vi "SQL_Search_Drivername.vi"(6 "Client Name (MSOLEDBSQL)":string="MSOLEDBSQL", 8 "error in (no error)":errorcluster caption="Fehler (Eingang, kein Fehler)") -> (0 "error out":errorcluster caption="Fehler (Ausgang)", 1 "Driver":string[](array[string]) caption="Alle ODBC Driver", 2 "found?":bool, 3 "Client Name":string)   [LabVIEW 2024, in "DB-Tool.lvlib"]
doc: "Es wird in der Windows-Registry nach dem angegebenen SQL-OLEDB-Provider gesucht.\nStandardmäßig wird nach \"<b>MSOLEDBSQL</b>\" gesucht, um einen installierten Microsoft SQL Server OLE DB Treiber zu finden.\n\n<b>Wichtig:</b>\nDer <b>SQL Server Native Client (SQLNCLI)</b> gilt als veraltet und sollte für neue Projekte nicht mehr verwendet werden.\nMicrosoft empfiehlt für Neuentwicklungen den aktuellen <b>Microsoft OLE DB Driver for SQL Server (MSOLEDBSQL)</b>.\n\n\nDer aktuelle Treiber kann hier heruntergeladen werden:\nhttps://learn.microsoft.com/en-us/sql/connect/oledb/download-oledb-driver-for-sql-server?view=sql-server-ver17\nMicrosoft OLE DB Driver for SQL Server herunterladen\n\nDas VI durchsucht die Registry nach verfügbaren SQL-OLEDB-Treibern und liefert den gefundenen Providernamen zurück.\nDadurch kann die Anwendung verschiedene installierte Treiberversionen automatisch erkennen, Beispielsweise: \n MSOLEDBSQL\n MSOLEDBSQL18\n MSOLEDBSQL19\n\nWird kein passender Treiber gefunden, wird der Ausgang <b>found?</b> auf FALSE gesetzt.\n\nEingänge:\n- Client Name: Name des gesuchten SQL/OLEDB-Clients (Standard wird nach MSOLEDBSQL gesucht).\n- error in: Hat keinen Einfluss über die Funktion.\n\nAusgänge:\n- Driver: Gefundener Treibername.\n- found?: TRUE, wenn ein passender Treiber gefunden wurde."
uses:
  <vilib>/registry/registry.llb/Registry RtKey.ctl
  <vilib>/registry/registry.llb/Registry SAM.ctl
  <vilib>/regexp/Match Regular Expression.xnode
  DB-Tool.lvlib
panel:
  # "Alt, sollte nicht mehr verwendet werden\nSQL Server Native Client\n\nNeu MSOLEDBSQL \n(sucht nach dem Treiber z.b. MSOLEDBSQL19.1)"
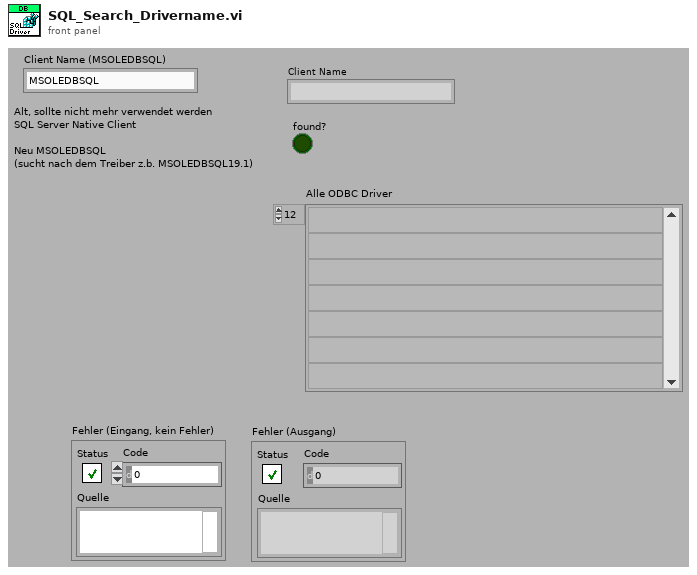
[diagram p1: front panel]
types:
  T1 = typedef "Registry SAM.ctl" = enum32{"KEY_QUERY_VALUE", "KEY_SET_VALUE", "KEY_CREATE_SUB_KEY", "KEY_ENUMERATE_SUB_KEYS", "KEY_NOTIFY", "KEY_CREATE_LINK", "KEY_READ", "KEY_WRITE", "KEY_ALL_ACCESS", "KEY_READ | KEY_WRITE"}
  T2 = typedef "Registry RtKey.ctl" = enum32{"HKEY_CLASSES_ROOT", "HKEY_CURRENT_USER", "HKEY_LOCAL_MACHINE", "HKEY_USERS", "HKEY_PERFORMANCE_DATA", "HKEY_CURRENT_CONFIG", "HKEY_DYN_DATA"}
  T3 = typedef "Registry refnum.ctl" = refnum<k1>
  T4 = cluster{"numSubKeys":i32, "maxSubKeyLen":i32, "maxSubKeyClassLen":i32}
  T5 = cluster{"numValues":i32, "maxValueNameLen":i32, "maxValueDataLen":i32}
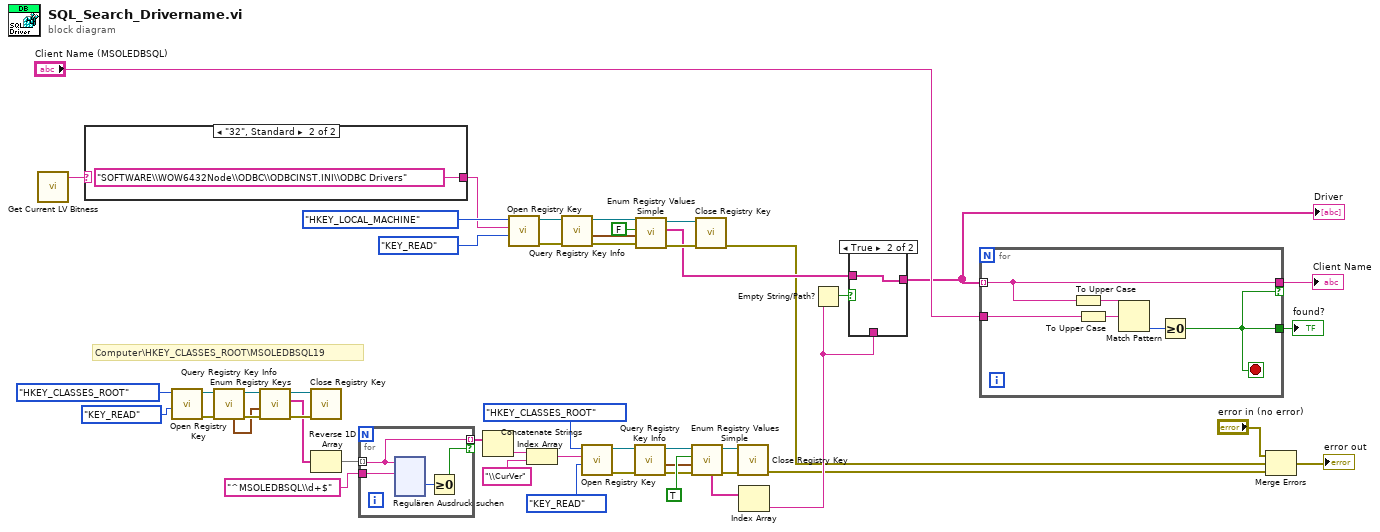
[diagram p0: block diagram]
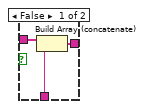
[diagram p2: hidden frame]
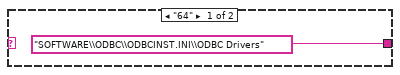
[diagram p3: hidden frame]
diagram:
  # "Computer\\HKEY_CLASSES_ROOT\\MSOLEDBSQL19"
  n1 = call <vilib>:"Get Current LV Bitness.vi"() -> ("bitness"=w45:string)  [unwired: 11 in]
  n2 = case shown="\"32\", Standard" w45 {
    tunnel: ["SOFTWARE\\ODBC\\ODBCINST.INI\\ODBC Drivers" ("subkey") "SOFTWARE\\WOW6432Node\\ODBC\\ODBCINST.INI\\ODBC Drivers" ("subkey")] -> w31
    frame "64" {
    }
    frame "32", Default {
    }
  }
  n3 = call <vilib>:"Open Registry Key.vi"("security access mask (KEY_READ | KEY_WRITE)"=Registry_SAM."KEY_READ", "root key (HKEY_LOCAL_MACHINE)"=Registry_RtKey."HKEY_CLASSES_ROOT") -> ("error out"=w33:errorcluster, "refnum out"=w35:T3)  [unwired: 8 in]
  n4 = call <vilib>:"Query Registry Key Info.vi"("error in (no error)"=w33, "refnum"=w35) -> ("error out"=w28:errorcluster, "refnum out"=w21:T3, "subkey info"=w22:T4)  [unwired: 5 in, 2 out]
  n5 = call <vilib>:"Enum Registry Keys.vi"("error in (no error)"=w28, "subkey info"=w22, "refnum"=w21) -> ("error out"=w30:errorcluster, "subkeys"=w27:string[], "refnum out"=w20:T3)  [unwired: 6 in]
  n6 = call <vilib>:"Close Registry Key.vi"("error in (no error)"=w30, "refnum"=w20) -> ()  [unwired: 5 in, 1 out]
  n7 = Reverse 1D Array(array=w27) -> (reversed array=w26:string[])
  n8 = for {
    tunnel: w26 -> [w55] mode=indexing
    tunnel: [w55] -> w25 mode=indexing if=w54
    tunnel: "^MSOLEDBSQL\\d+$" ("Regulärer Ausdruck") -> [w53]
    n9 = xnode "Regulären Ausdruck suchen"("Eingangs-String"=w55, "Regulärer Ausdruck"=w53) -> ("Offset nach Übereinstimmung"=w56:i32)  [unwired: 4 in, 4 out]
    n10 = Greater Or Equal To 0?(x=w56) -> (x >= 0?=w54:bool)
  }
  n11 = Index Array(array=w25) -> (element=w8:string)  [unwired: 1 in]
  n12 = call <vilib>:"Open Registry Key.vi"("security access mask (KEY_READ | KEY_WRITE)"=Registry_SAM."KEY_READ", "subkey"=w31, "root key (HKEY_LOCAL_MACHINE)"=Registry_RtKey."HKEY_LOCAL_MACHINE") -> ("error out"=w41:errorcluster, "refnum out"=w37:T3)  [unwired: 7 in]
  n13 = Concatenate Strings(w8, "\\CurVer" ("String")) -> (w7:string)
  n14 = call <vilib>:"Query Registry Key Info.vi"("error in (no error)"=w41, "refnum"=w37) -> ("error out"=w42:errorcluster, "value info"=w36:T5, "refnum out"=w29:T3)  [unwired: 5 in, 2 out]
  n15 = call <vilib>:"Open Registry Key.vi"("security access mask (KEY_READ | KEY_WRITE)"=Registry_SAM."KEY_READ", "subkey"=w7, "root key (HKEY_LOCAL_MACHINE)"=Registry_RtKey."HKEY_CLASSES_ROOT") -> ("error out"=w18:errorcluster, "refnum out"=w16:T3)  [unwired: 7 in]
  n16 = call <vilib>:"Query Registry Key Info.vi"("error in (no error)"=w18, "refnum"=w16) -> ("error out"=w9:errorcluster, "value info"=w13:T5, "refnum out"=w15:T3)  [unwired: 5 in, 2 out]
  n17 = call <vilib>:"Enum Registry Values Simple.vi"("error in (no error)"=w42, "value info"=w36, "retrieve data? (F)"=FALSE, "refnum"=w29) -> ("error out"=w40:errorcluster, "values"=w24:string[], "refnum out"=w39:T3)  [unwired: 2 in, 3 out]
  n18 = call <vilib>:"Enum Registry Values Simple.vi"("error in (no error)"=w9, "value info"=w13, "retrieve data? (F)"=TRUE, "refnum"=w15) -> ("error out"=w10:errorcluster, "refnum out"=w11:T3, "String/Binary data"=w12:string[])  [unwired: 2 in, 3 out]
  n19 = call <vilib>:"Close Registry Key.vi"("error in (no error)"=w40, "refnum"=w39) -> ("error out"=w2:errorcluster)  [unwired: 5 in]
  n20 = call <vilib>:"Close Registry Key.vi"("error in (no error)"=w10, "refnum"=w11) -> ("error out"=w1:errorcluster)  [unwired: 5 in]
  n21 = Index Array(array=w12) -> (element=w4:string)  [unwired: 1 in]
  n22 = Empty String/Path?(string/path=w4) -> (empty?=w3:bool)
  n23 = case shown="True" w3 {
    tunnel: w24 -> [w176 w177]
    tunnel: [w175 w177] -> w5
    tunnel: w4 -> [w174 _]
    frame False {
      n24 = Build Array (concatenate)(w176, w174) -> (w175:string[])
    }
    frame True {
    }
  }
  "Driver" <- w5
  n25 = for {
    tunnel: w5 -> [w180] mode=indexing
    tunnel: [w180] -> w50 if=w178
    tunnel: [w178] -> w47
    tunnel: "Client Name (MSOLEDBSQL)" -> [w179]
    stop <- w178 stop-if-true
    n26 = To Upper Case(1:w180) -> (0:w182:string)
    n27 = To Upper Case(1:w179) -> (0:w183:string)
    n28 = Match Pattern(string=w182, regular expression=w183) -> (offset past match=w181:i32)  [unwired: 1 in, 3 out]
    n29 = Greater Or Equal To 0?(x=w181) -> (x >= 0?=w178:bool)
  }
  "Client Name" <- w50
  "found?" <- w47
  n30 = Merge Errors("error in (no error)", w2, w1) -> (→"error out":errorcluster)
